vi "Scheduler_Claim_Resources.vi"(8 "error in (no error)":errorcluster={"status"=FALSE, "code"=0, "source"="\"\""}, 10 "lease table":string, 11 "Ready step resource declarations":string) -> (0 "error out":errorcluster={"status"=FALSE, "code"=0, "source"="\"\""}, 2 "status ok":bool, 3 "Ownership tokens or busy state":string)   [LabVIEW 2026]
doc: "INTENT: Reserve command resources for action. LOGIC: Request all required leases in stable sorted order; reject/serialize conflicts before commanding."
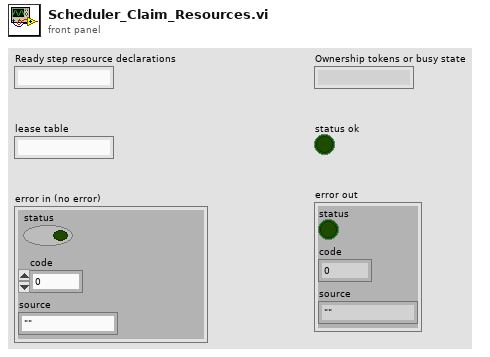
[diagram p1: front panel]
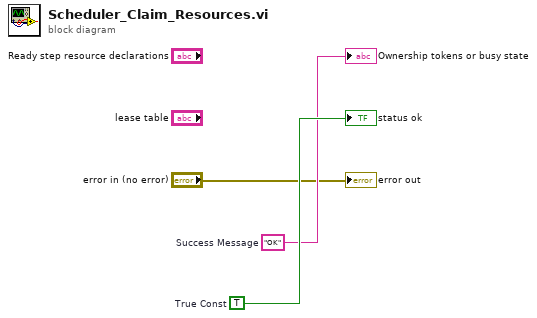
[diagram p0: block diagram]
diagram:
  w3 = TRUE  # True Const
  w2 = "OK"  # Success Message
  "Ownership tokens or busy state" <- w2
  "status ok" <- w3
  "error out" <- "error in (no error)"
